vi "MeaAll.vi"() -> ()   [LabVIEW 2015]
panel:
  out "数据缓存":u8[](array[numeric])
  out "data_out":sgl[](array[numeric])
  out "解析后的字符串":string
  in  "读取的字节数":u32=400
  out "Dll路径":path
  in  "超时(ms)":u32=2000
  in  "设备地址":string="[C:DSO][D:DSO-X][T:USB][PID:0x5537][VID:0x4348][EI:0x82][EO:0x2][CFG:1][I:0]"
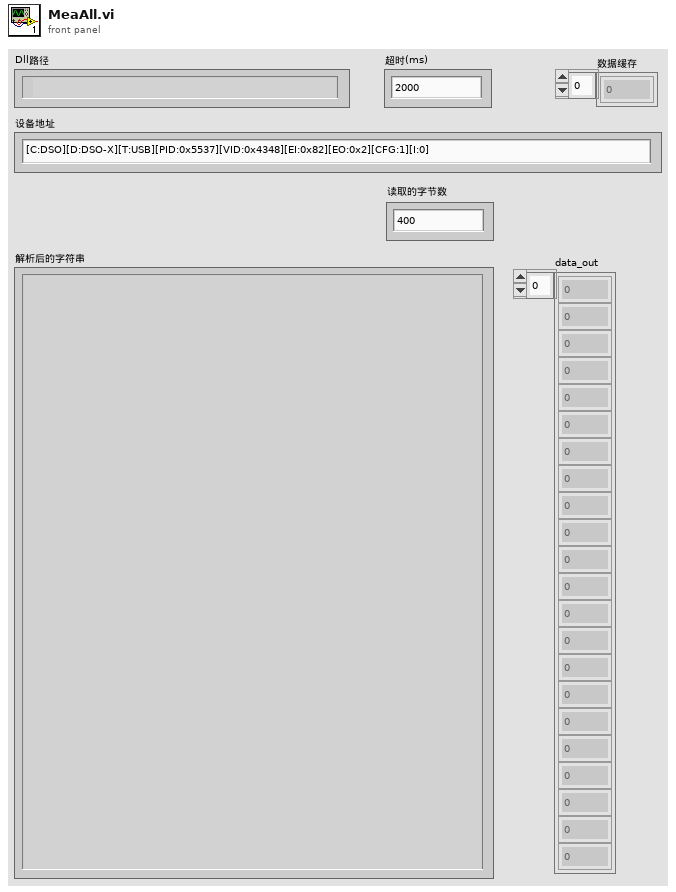
[diagram p1: front panel]
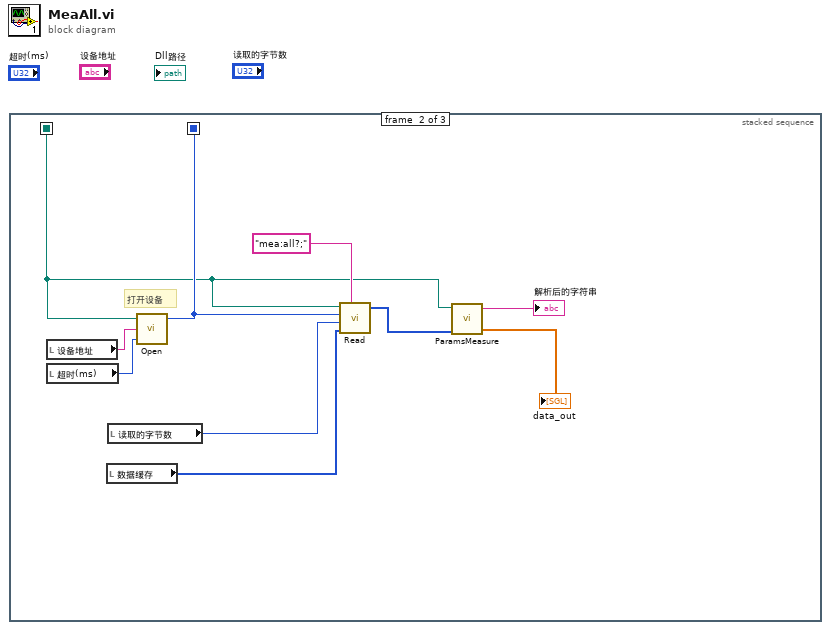
[diagram p0: block diagram]
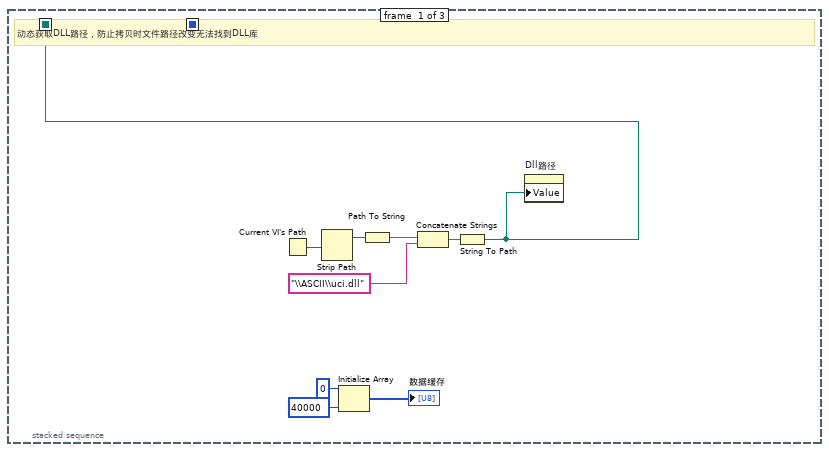
[diagram p2: hidden frame]
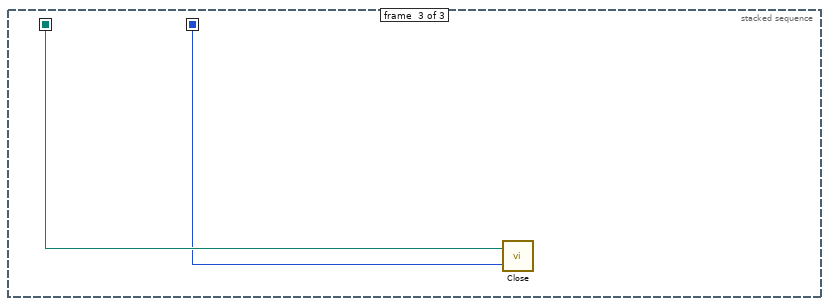
[diagram p3: hidden frame]
diagram:
  n1 = stacked-sequence {
    seq-local: [w4 _ _] -> [_ w14 w21]
    seq-local: [_ w16 _] -> [_ _ w20]
    frame #0 {
      # "动态获取DLL路径，防止拷贝时文件路径改变无法找到DLL库"
      n2 = Current VI's Path() -> (path=w8:path)
      n3 = Strip Path(path=w8) -> (stripped path=w6:path)  [unwired: 1 out]
      n4 = Initialize Array(u8 0 ("元素"), 40000 ("维数大小")) -> (→"数据缓存":u8[])
      n5 = Path To String(path=w6) -> (string=w5:string)
      n6 = Concatenate Strings(w5, "\\ASCII\\uci.dll" ("字符串")) -> (w7:string)
      n7 = String To Path(string=w7) -> (path=w4:path)
      n8 = property on="Dll路径" class="Path"("Value"=w4) -> ()  [unwired: 2 in, 2 out]
    }
    frame #1 {
      # "打开设备"
      n9 = local read "设备地址"() -> (w19:string)
      n10 = local read "超时(ms)"() -> (w17:u32)
      n11 = local read "数据缓存"() -> (w10:u8[])
      n12 = local read "读取的字节数"() -> (w18:u32)
      n13 = call "Open.vi"("Timeout"=w17, "Addr"=w19, "UCI_DllPath"=w14) -> ("Session_id"=w16:i32)  [unwired: 2 out]
      n14 = call "Read.vi"("UCI_DllPath"=w14, "Command"="mea:all?;" ("指令"), "Session_id"=w16, "Length"=w18, "InputData"=w10) -> ("OutputData"=w13:u8[])  [unwired: 1 in, 2 out]
      n15 = call "ParamsMeasure.vi"("InputData"=w13, "UCI_DllPath"=w14) -> ("OuputData"=→"data_out":sgl[], "OutputString"=→"解析后的字符串":string)  [unwired: 3 in]
    }
    frame #2 {
      n16 = call "Close.vi"("Session_id"=w20, "UCI_DllPath"=w21) -> ()  [unwired: 1 out]
    }
  }
